vi "query Operation Band.vi"(8 "error in (no error)":errorcluster, 10 "Selected CC Argements":T1, 11 "NR in":refnum<class "NR.lvclass">) -> (0 "error out":errorcluster, 2 "Operation Band":u32, 3 "NR out":refnum<class "NR.lvclass">)   [LabVIEW 2023, in "ANRITSU Call Box.lvlib" / "NR.lvclass"]
uses:
  NR.lvclass
  NR.lvclass/NR.ctl
  ANRITSU Call Box.lvlib
  Type Definition/NR Selected CC Type Arguments.ctl
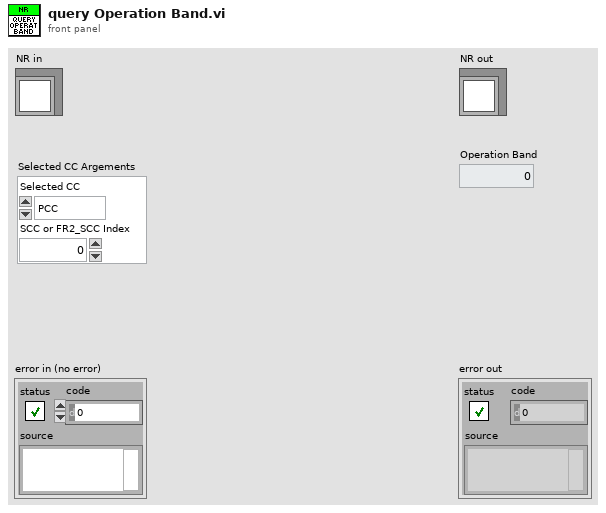
[diagram p1: front panel]
types:
  T1 = typedef "ANRITSU Call Box.lvlib/NR Selected CC Type Arguments.ctl" = cluster{"Selected CC":enum16{"PCC", "SCC", "FR2_PCC", "FR2_SCC"}, "SCC or FR2_SCC Index":u32}
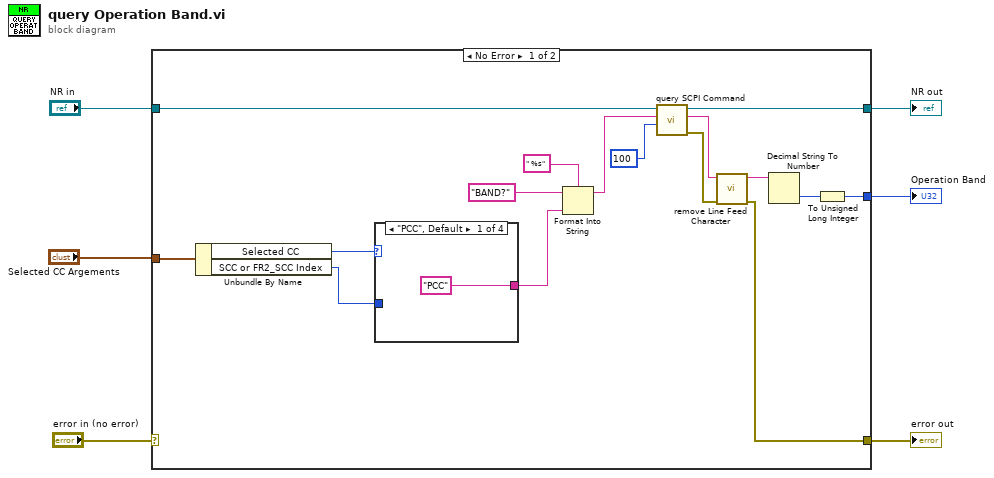
[diagram p0: block diagram]
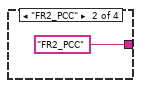
[diagram p2: hidden frame]
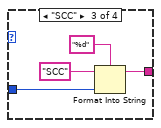
[diagram p3: hidden frame]
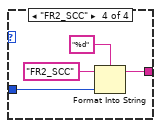
[diagram p4: hidden frame]
diagram:
  n1 = case shown="No Error" "error in (no error)" {
    selector: "error in (no error)" -> [_ w33]
    tunnel: "NR in" -> [w16 w34]
    tunnel: [w13 w34] -> w5
    tunnel: [w7 w33] -> w4
    tunnel: "Selected CC Argements" -> [w22 _]
    tunnel: [w8 _] -> w1
    frame No Error {
      n2 = Unbundle By Name(w22) -> ("Selected CC"=w21:enum16{"PCC", "SCC", "FR2_PCC", "FR2_SCC"}, "SCC or FR2_SCC Index"=w20:u32)
      n3 = case shown="\"PCC\", Default" w21 {
        tunnel: ["PCC" "FR2_PCC" w25 w29] -> w18
        tunnel: w20 -> [_ _ w26 w30]
        frame "PCC", Default {
        }
        frame "FR2_PCC" {
        }
        frame "SCC" {
          n4 = Format Into String(format string="%d", initial string="SCC", w26) -> (resulting string=w25:string)  [unwired: 1 in, 1 out]
        }
        frame "FR2_SCC" {
          n5 = Format Into String(format string="%d", initial string="FR2_SCC", w30) -> (resulting string=w29:string)  [unwired: 1 in, 1 out]
        }
      }
      n6 = Format Into String(format string=" %s", initial string="BAND?", w18) -> (resulting string=w15:string)  [unwired: 1 in, 1 out]
      n7 = call "query SCPI Command.vi"("Read Buffer Length"=u32 100, "SCPI Command"=w15, "NR in"=w16) -> ("error out"=w11:errorcluster, "Read Buffer String"=w12:string, "NR out"=w13:refnum<class "NR.lvclass">)  [unwired: 6 in]
      n8 = call "remove Line Feed Character.vi"("error in"=w11, "Query String"=w12) -> ("error out"=w7:errorcluster, "Line Feed Removed String"=w9:string)  [unwired: 8 in]
      n9 = Decimal String To Number(string=w9) -> (number=w10:i32)  [unwired: 2 in, 1 out]
      n10 = To Unsigned Long Integer(number=w10) -> (unsigned 32bit integer=w8:u32)
    }
    frame Error {
    }
  }
  "error out" <- w4
  "NR out" <- w5
  "Operation Band" <- w1
